vi "Cleanup.vi"(8 "error in (no error)":errorcluster, 11 "PanelArray in":refnum<class "ArrayManager.lvclass">) -> (0 "error out":errorcluster)   [LabVIEW 2020, in "OOPanel.lvlib" / "ArrayManager.lvclass"]
uses:
  ArrayManager.lvclass
  ArrayManager.lvclass/ArrayManager.ctl
  Manager/Manager.lvclass
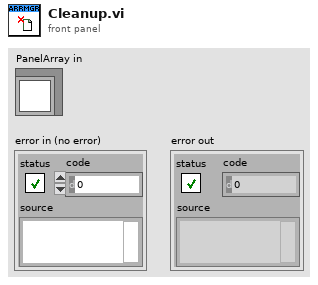
[diagram p1: front panel]
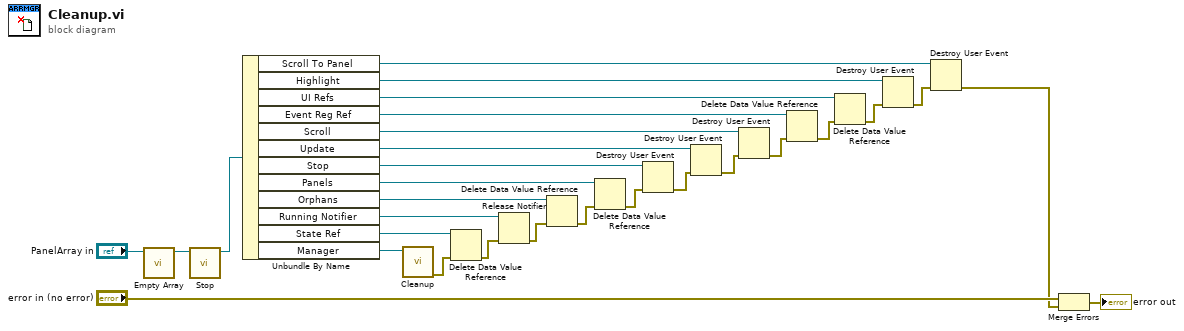
[diagram p0: block diagram]
diagram:
  n1 = call "Empty Array.vi"("ArrayManager in"="PanelArray in") -> ("ArrayManager out"=w6:refnum<class "ArrayManager.lvclass">)  [unwired: 9 in, 1 out]
  n2 = call "Stop.vi"("ArrayManager in"=w6) -> ("ArrayManager out"=w25:refnum<class "ArrayManager.lvclass">)  [unwired: 9 in, 1 out]
  n3 = Unbundle By Name(w25) -> ("Scroll To Panel"=w3:refnum<user-event>, "Highlight"=w5:refnum<user-event>, "UI Refs"=w8:refnum<data-value>, "Event Reg Ref"=w10:refnum<data-value>, "Scroll"=w11:refnum<user-event>, "Update"=w14:refnum<user-event>, "Stop"=w16:refnum<user-event>, "Panels"=w19:refnum<data-value>, "Orphans"=w20:refnum<data-value>, "Running Notifier"=w22:refnum<notifier>, "State Ref"=w24:refnum<data-value>, "Manager"=w28:refnum<class "Manager.lvclass">)
  n4 = call "Cleanup.vi"("Manager in"=w28) -> ("error out"=w23:errorcluster)  [unwired: 8 in, 2 out]
  n5 = Delete Data Value Reference(data value reference=w24, error in=w23) -> (error out=w21:errorcluster)  [unwired: 1 out]
  n6 = Release Notifier(notifier=w22, error in (no error)=w21) -> (error out=w18:errorcluster)  [unwired: 1 in, 2 out]
  n7 = Delete Data Value Reference(data value reference=w20, error in=w18) -> (error out=w17:errorcluster)  [unwired: 1 out]
  n8 = Delete Data Value Reference(data value reference=w19, error in=w17) -> (error out=w15:errorcluster)  [unwired: 1 out]
  n9 = Destroy User Event(user event=w16, error in=w15) -> (error out=w13:errorcluster)
  n10 = Destroy User Event(user event=w14, error in=w13) -> (error out=w12:errorcluster)
  n11 = Destroy User Event(user event=w11, error in=w12) -> (error out=w9:errorcluster)
  n12 = Delete Data Value Reference(data value reference=w10, error in=w9) -> (error out=w7:errorcluster)  [unwired: 1 out]
  n13 = Delete Data Value Reference(data value reference=w8, error in=w7) -> (error out=w4:errorcluster)  [unwired: 1 out]
  n14 = Destroy User Event(user event=w5, error in=w4) -> (error out=w2:errorcluster)
  n15 = Destroy User Event(user event=w3, error in=w2) -> (error out=w1:errorcluster)
  n16 = Merge Errors("error in (no error)", w1) -> (→"error out":errorcluster)
